vi "Ctor.vi"(8 "error in (no error)":errorcluster, 11 "DeviceListPanel in":refnum<class "DeviceListPanel.lvclass">) -> (0 "error out":errorcluster, 3 "DeviceListPanel out":refnum<class "DeviceListPanel.lvclass">)   [LabVIEW 2020, in "PicoG-App.lvlib" / "DeviceListPanel.lvclass"]
uses:
  DeviceListPanel.lvclass
  Ref Data.ctl
  Device/Device Key.ctl
  Device and Panel.ctl
  Device/Device.lvclass
  DeviceArrayPanel/DeviceArrayPanel.lvclass
  DeviceListPanel.lvclass/DeviceListPanel.ctl
  <vilib>/IlluminatedG/IG OOPanel/OOPanel/Panel/Panel.lvclass
  <vilib>/IlluminatedG/IG OOPanel/OOPanel/ArrayManager/ArrayManager.lvclass
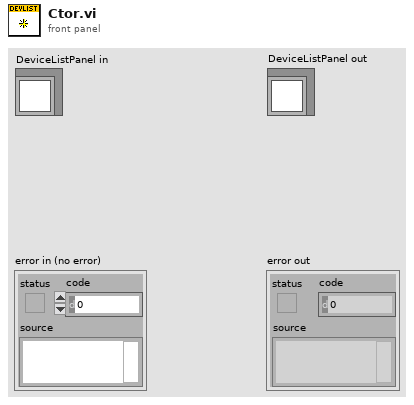
[diagram p1: front panel]
types:
  T1 = typedef "PicoG-App.lvlib/DeviceListPanel.lvclass/Ref Data.ctl" = cluster{"Map":map{T2, T3}}
  T2 = typedef "PicoG-App.lvlib/Device.lvclass/Device Key.ctl" = cluster{"Platform":string, "Board":string, "ID":string}
  T3 = typedef "PicoG-App.lvlib/DeviceListPanel.lvclass/Device and Panel.ctl" = cluster{"Device":refnum<class "Device.lvclass">, "Panel":refnum<class "DeviceArrayPanel.lvclass">}
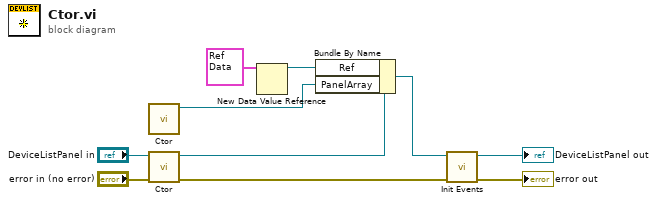
[diagram p0: block diagram]
diagram:
  n1 = call <vilib>:"Ctor.vi"() -> ("PanelArray"=w2:refnum<class "ArrayManager.lvclass">)  [unwired: 10 in, 1 out]
  n2 = call-parent <vilib>:"Ctor.vi"("error in (no error)"="error in (no error)", "Panel in"="DeviceListPanel in") -> ("error out"=w7:errorcluster, "Panel out"=w8:refnum<class "DeviceListPanel.lvclass">)  [unwired: 8 in]
  n3 = New Data Value Reference(data value=T1 {"Map"={}} ("Ref Data")) -> (data value reference=w3:refnum<data-value>)  [unwired: 1 in, 1 out]
  n4 = Bundle By Name(cluster=w8, "Ref"=w3, "PanelArray"=w2) -> (w4:refnum<class "DeviceListPanel.lvclass">)
  n5 = call "Init Events.vi"("error in (no error)"=w7, "DeviceListPanel in"=w4) -> ("error out"=→"error out":errorcluster, "DeviceListPanel out"=→"DeviceListPanel out":refnum<class "DeviceListPanel.lvclass">)  [unwired: 8 in]
